vi "Heat Flow Front Panel.vi"() -> ()   [LabVIEW 2019, in "Results.lvlib" / "Heat Flow Results.lvclass"]
uses:
  Heat Flow Results.lvclass
  Heat Flow Results.lvclass/Heat Flow Results.ctl
  Test Stands/Heat Flow/Heat Flow Test Stand.lvclass
panel:
  out "Htr H temp 2":dbl caption="Heater Hot Side Temperature, C" format="%.1f"
  out "Htr C temp 2":dbl caption="Heater Cold Side Temperature, C" format="%.1f"
  out "U Load 2":dbl caption="U Load, mV" format="%#.3f"
  out "P TEG 2":dbl caption="P TEG 2, mW" format="%#.3f"
  out "I Load 2":dbl caption="I Load, mA" format="%#.3f"
  out "R shunt":dbl
  out "U R htr":dbl caption="U R htr, V" format="%#.3f"
  out "U R shunt":dbl caption="U R shunt, V" format="%.3f"
  out "TEG C temp":dbl caption="TEG Cold Side Temperature" format="%#.2f"
  in  "R Load":dbl=48.0 caption="R Load, Ohm" min=0.0 max=1000.0 step=0.1 format="%#.3f"
  in  "Ugs Hot":dbl min=0.0 max=10.0 step=0.1
  out "TEG C temp":dbl caption="TEG Hot Side Temperature" format="%#.2f"
  out "Adjusted":bool
  in  "Heater Temp SP":dbl min=0.0 max=372.0 step=1.0
  in  "auto Temp":bool
  in  "Ugs Cold":dbl min=0.0 max=10.0 step=0.1
  in  "Heater Power SP":dbl min=0.0 max=300.0 step=1.0
  in  "auto pwr":bool
  out "Htr C temp":dbl caption="Heater Cold Side Temperature" format="%#.2f"
  out "Htr H temp":dbl caption="Heater Hot Side Temperature" format="%#.2f"
  out "U Load":dbl caption="U Load, V" format="%#.6f"
  out "P Heater":dbl caption="P Heater, W" format="%#.3f"
  out "I Heater":dbl caption="I Heater, A" format="%.3f"
  out "I Load":dbl caption="I Load, A" format="%#.3f"
  out "P TEG":dbl format="%#.4f"
  # "G-M\nCryocooler"
  # "Automatic"
  # "24 V"
  # "Manual"
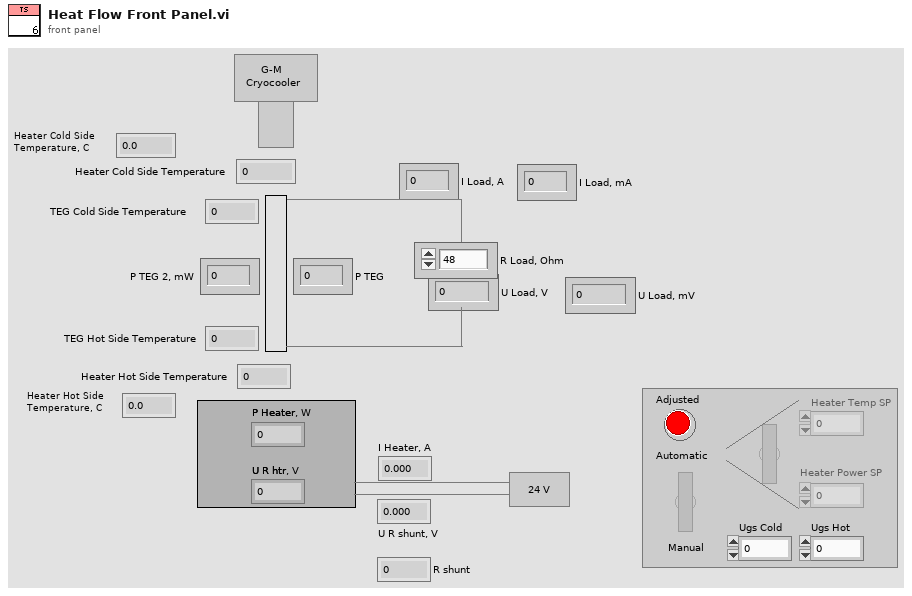
[diagram p1: front panel]
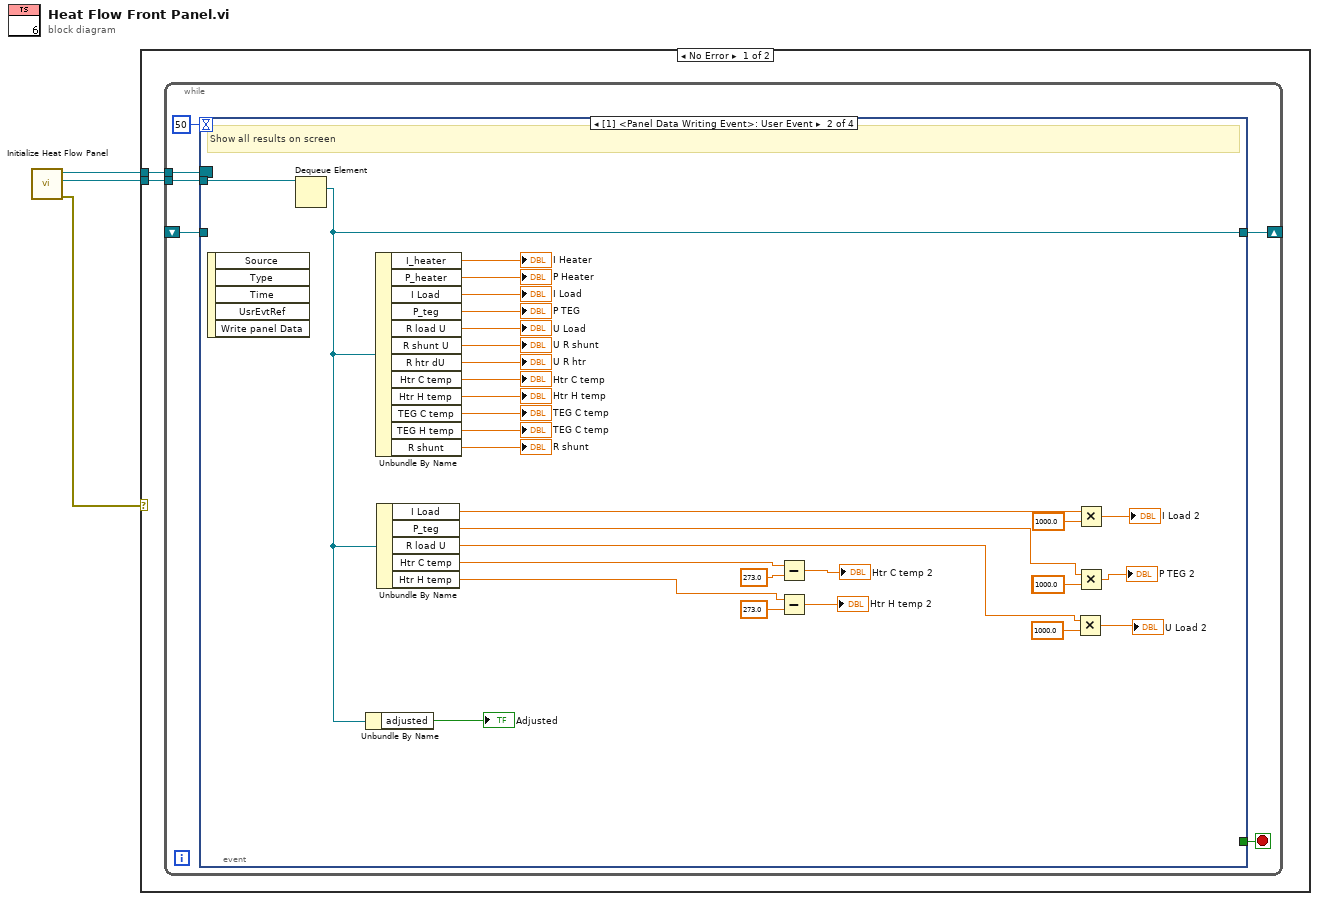
[diagram p0: block diagram]
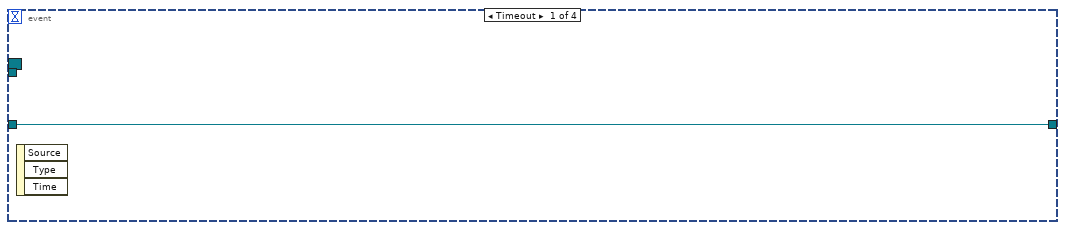
[diagram p2: hidden frame]
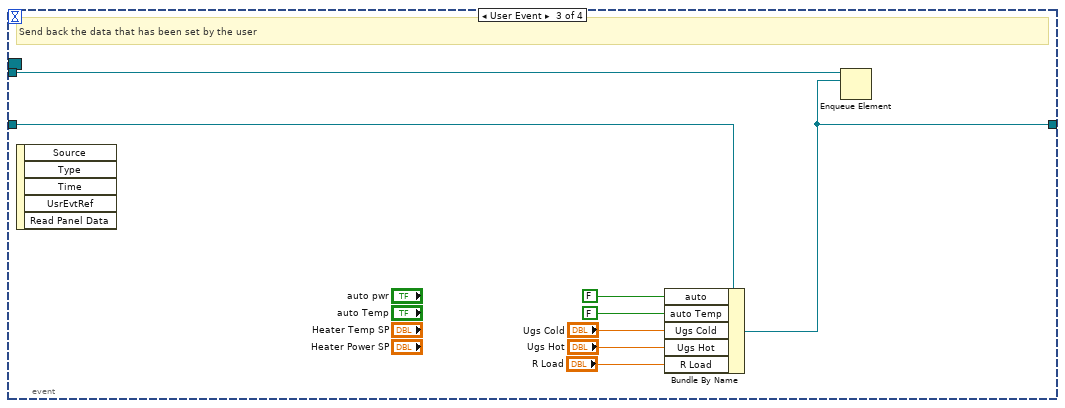
[diagram p3: hidden frame]
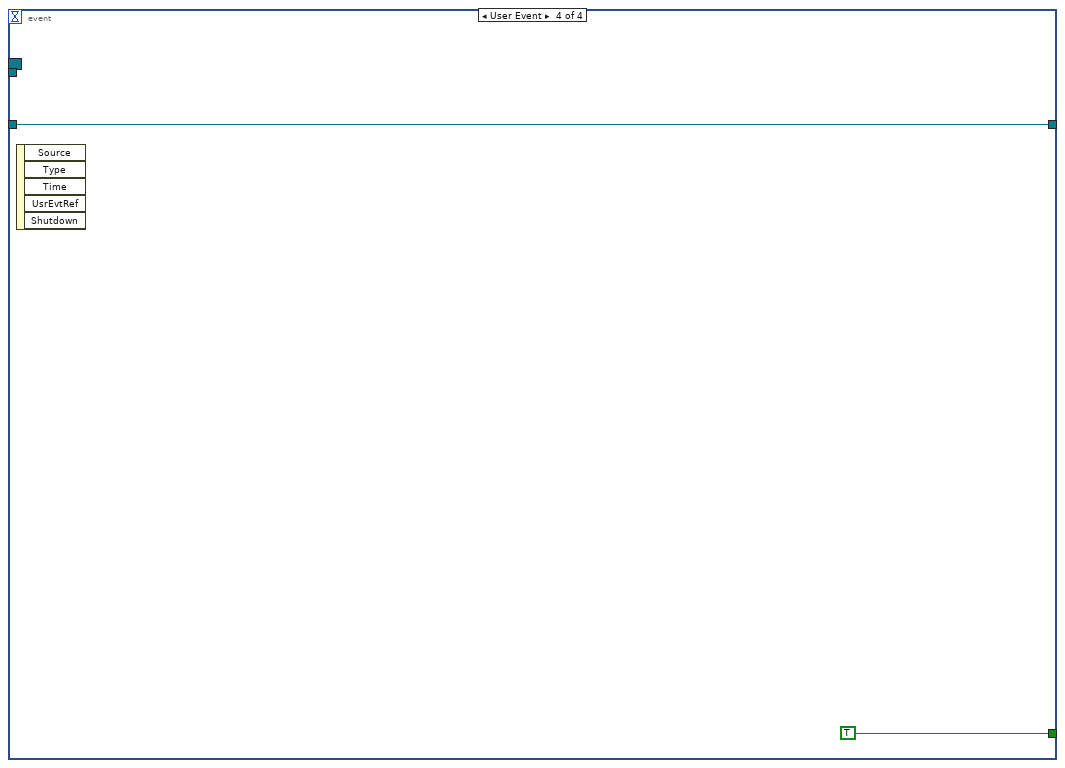
[diagram p4: hidden frame]
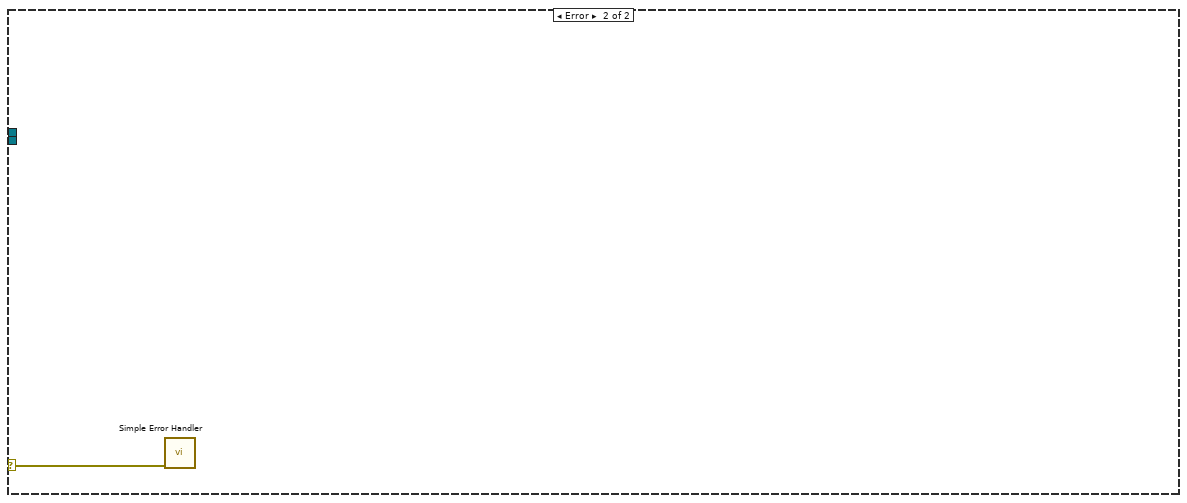
[diagram p5: hidden frame]
diagram:
  n1 = call "Initialize Heat Flow Panel.vi"() -> ("error out"=w3:errorcluster, "Heat Flow Results queue out"=w1:refnum<queue>, "Event Registration Refnum"=w2:refnum<event-registration>)  [unwired: 9 in]
  n2 = case shown="No Error" w3 {
    selector: w3 -> [_ w53]
    tunnel: w2 -> [w5 _]
    tunnel: w1 -> [w4 _]
    frame No Error {
      n3 = while {
        tunnel: w5 -> [w10]
        tunnel: w4 -> [w9]
        shift-right: [w7] -> _
        shift-left: _ -> [w6]
        stop <- w11 stop-if-true
        n4 = event shown="[1] <Panel Data Writing Event>: User Event" {
          selector: w10 -> [_ _ _ _]
          dyn-events: _ -> [_ _ _ _]
          timeout: 50 -> [_ _ _ _]
          tunnel: [_ _ _ TRUE] -> w11
          tunnel: w9 -> [_ w42 w50 _]
          tunnel: [w12 w28 w48 w51] -> w7
          tunnel: w6 -> [w12 _ w49 w51]
          event Timeout {
            n5 = event-data() -> ()  [unwired: 1 in, 3 out]
          }
          event User Event {
            (unwired) 1000.0 ("y")
            # "Show all results on screen"
            n6 = event-data() -> ()  [unwired: 1 in, 5 out]
            n7 = Dequeue Element(queue=w42) -> (element=w28:refnum<class "Heat Flow Results.lvclass">)  [unwired: 2 in, 3 out]
            n8 = Unbundle By Name(w28) -> ("adjusted"=→"Adjusted":bool)
            n9 = Unbundle By Name(w28) -> ("I_heater"=→"I Heater":dbl, "P_heater"=→"P Heater":dbl, "I Load"=→"I Load":dbl, "P_teg"=→"P TEG":dbl, "R load U"=→"U Load":dbl, "R shunt U"=→"U R shunt":dbl, "R htr dU"=→"U R htr":dbl, "Htr C temp"=→"Htr C temp":dbl, "Htr H temp"=→"Htr H temp":dbl, "TEG C temp"=→"TEG C temp":dbl, "TEG H temp"=→"TEG C temp":dbl, "R shunt"=→"R shunt":dbl)
            n10 = Unbundle By Name(w28) -> ("I Load"=w27:dbl, "P_teg"=w13:dbl, "R load U"=w22:dbl, "Htr C temp"=w19:dbl, "Htr H temp"=w15:dbl)
            n11 = Subtract(x=w19, y=273.0) -> (x-y=→"Htr C temp 2":dbl)
            n12 = Subtract(x=w15, y=273.0) -> (x-y=→"Htr H temp 2":dbl)
            n13 = Multiply(x=w22, y=1000.0) -> (x*y=→"U Load 2":dbl)
            n14 = Multiply(x=w27, y=1000.0) -> (x*y=→"I Load 2":dbl)
            n15 = Multiply(x=w13, y=1000.0) -> (x*y=→"P TEG 2":dbl)
          }
          event User Event {
            # "Send back the data that has been set by the user"
            n16 = event-data() -> ()  [unwired: 1 in, 5 out]
            n17 = Bundle By Name(cluster=w49, "auto"=FALSE, "auto Temp"=FALSE, "Ugs Cold"="Ugs Cold", "Ugs Hot"="Ugs Hot", "R Load"="R Load") -> (w48:refnum<class "Heat Flow Results.lvclass">)
            n18 = Enqueue Element(queue=w50, element=w48) -> ()  [unwired: 2 in, 3 out]
          }
          event User Event {
            n19 = event-data() -> ()  [unwired: 1 in, 5 out]
          }
        }
      }
    }
    frame Error {
      n20 = call <vilib>:"Simple Error Handler.vi"("error in (no error)"=w53) -> ()  [unwired: 4 in, 5 out]
    }
  }
